vi "Main.vi"() -> ()   [LabVIEW 2013]
doc: "This template is for the Queued Message Handler design pattern.\n\nThe Event Handling Loop generates messages based on user interface actions.\n\nThe Message Handling Loop processes messages generated by the Event Handling Loop, or by other messages. The messages are string values, so new messages can be added easily to the Message Cases case structure in the Message Handling Loop. Each message cluster can also provide an optional value for Message Data, which is a variant that can be converted to whatever message-specific data is required."
uses:
  controls/UI Data.ctl
  <vilib>/vision/Image Controls.llb/IMAQ Image.ctl
  support/Message Queue/Message Queue.lvlib
  support/User Event - Stop/User Event - Stop.lvlib
  support/FPGA/FPGA Frame Grabbing.lvlib
  <vilib>/vision/NI_Vision_Development_Module.lvlib
  support/Image Processing/Image Processing.lvlib
panel:
  out "Wingbeat Amplitude Graph":dynamicdata(graph)
  in  "Stop Charts":bool
  in  "NumWingSectors":u8=12
  in  "Wing ROIs":T1
  out "combo mask":T2(plugin-control)
  out "right \nannulus":T3={"Center X"=1090, "Center Y"=659, "Inner Radius"=200, "Outer Radius"=405, "Start Angle"=0.0, "End Angle"=90.0} {"End Angle" format="%.2f"; "Start Angle" format="%.2f"; "Center X" scale=0.0..1024.0}
  out "right masked image":T2(plugin-control)
  out "right mask":T2(plugin-control)
  out "left annulus":T3={"Center X"=929, "Center Y"=663, "Inner Radius"=200, "Outer Radius"=405, "Start Angle"=90.0, "End Angle"=180.0} {"End Angle" format="%.2f"; "Start Angle" format="%.2f"; "Center X" scale=0.0..1024.0}
  out "left masked image":T2(plugin-control)
  out "left mask":T2(plugin-control)
  in  "Accept Threshold":bool
  in  "Threshold Range":cluster{"Lower value":dbl, "Upper value":dbl}={"Lower value"=106.82432432432432, "Upper value"=255.0} {"Upper value" min=0.0 max=255.0 scale=0.0..255.0; "Lower value" min=0.0 max=255.0 scale=0.0..255.0}
  out "FPGA image info":T6={"Image Type"=0, "Unit"=enum."Undefined", "X Resolution"=2040, "Y Resolution"=1088, "X Step"=1.0, "Y Step"=1.0, "Image Name"="Image"} {"Image Type" items=["Grayscale (U8)", "Grayscale (I16)", "Grayscale (SGL)", "Complex (CSG)", "RGB (U32)", "HSL (U32)", "RGB (U64)", "Grayscale (U16)"]}
  out "Processed Image":T2(plugin-control)
  in  "Stream?":bool
  out "FPGA Image":T2(plugin-control)
  in  "Save Mask Coordinates":bool
  in  "Test Visual Response":bool
  in  "Test FPGA":bool
  out "Status Update":string="VI Stopped"
  in  "Define Mask":bool
  in  "Acquire Image":bool
  in  "Stop":bool
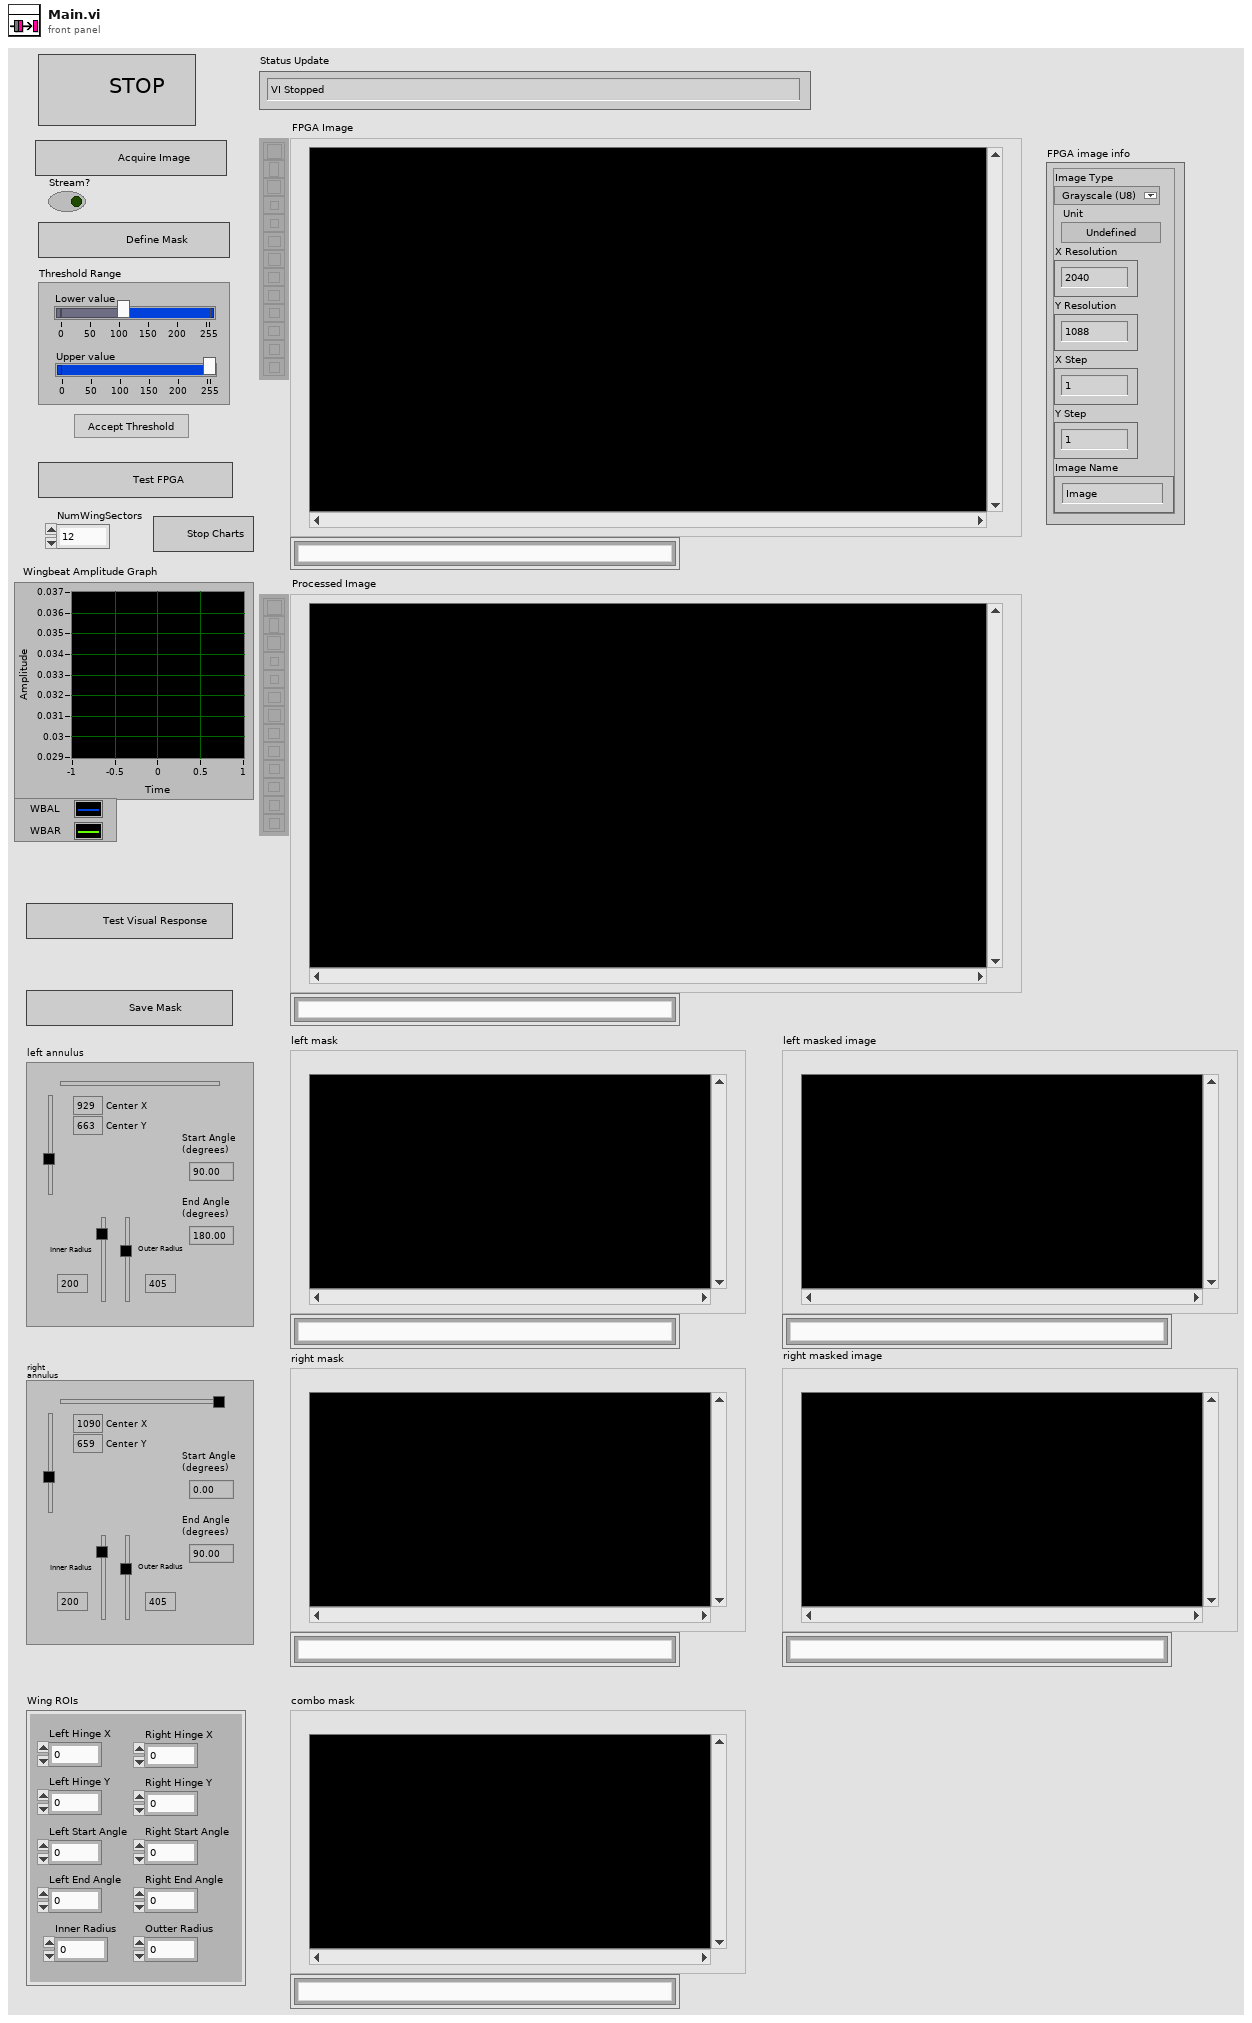
[diagram p1: front panel]
types:
  T1 = cluster{"Left Hinge X":u16, "Left Hinge Y":u16, "Inner Radius":u16, "Outter Radius":u16, "Right Hinge X":u16, "Right Hinge Y":u16, "Right Start Angle":i16, "Right End Angle":i16, "Left Start Angle":i16, "Left End Angle":i16}
  T2 = typedef "IMAQ Image.ctl" = refnum<image>
  T3 = typedef "IMAQ Circle" = cluster{"Center X":i32, "Center Y":i32, "Inner Radius":i32, "Outer Radius":i32, "Start Angle":dbl, "End Angle":dbl}
  T4 = typedef "Image Type" = u32
  T5 = typedef "Image Unit" = enum32{"Undefined", "Angström", "Micrometer", "Millimeter", "Centimeter", "Meter", "Kilometer", "Microinch", "Inch", "Feet", "Nautical miles", "Standard miles", "Steps"}
  T6 = cluster{"Image Type":T4, "Unit":T5, "X Resolution":i32, "Y Resolution":i32, "X Step":sgl, "Y Step":sgl, "Image Name":string}
  T7 = typedef "UI Data.ctl" = cluster{"Boolean <Replace Me>":bool, "Initial Message":string, "Numeric <Replace Me>":dbl, "Acquire Image Ref":refnum<vi>, "Define Mask Ref":refnum<vi>, "Status Update Ref":refnum<vi>, "Stop Button Ref":refnum<vi>, "FPGA Image":T2, "Processed Image":T2, "Left Annulus":cluster{"Center X":i32, "Center Y":i32, "Inner Radius":i32, "Outer Radius":i32, "Start Angle":dbl, "End Angle":dbl}, "Right Annulus":cluster{"Center X":i32, "Center Y":i32, "Inner Radius":i32, "Outer Radius":i32, "Start Angle":dbl, "End Angle":dbl}}
  T8 = typedef "Message Queue.lvlib/All Message Queues.ctl" = cluster{"UI":refnum<queue>}
  T9 = cluster{"Center X":i32, "Center Y":i32, "Inner Radius":i32, "Outer Radius":i32, "Start Angle":dbl, "End Angle":dbl}
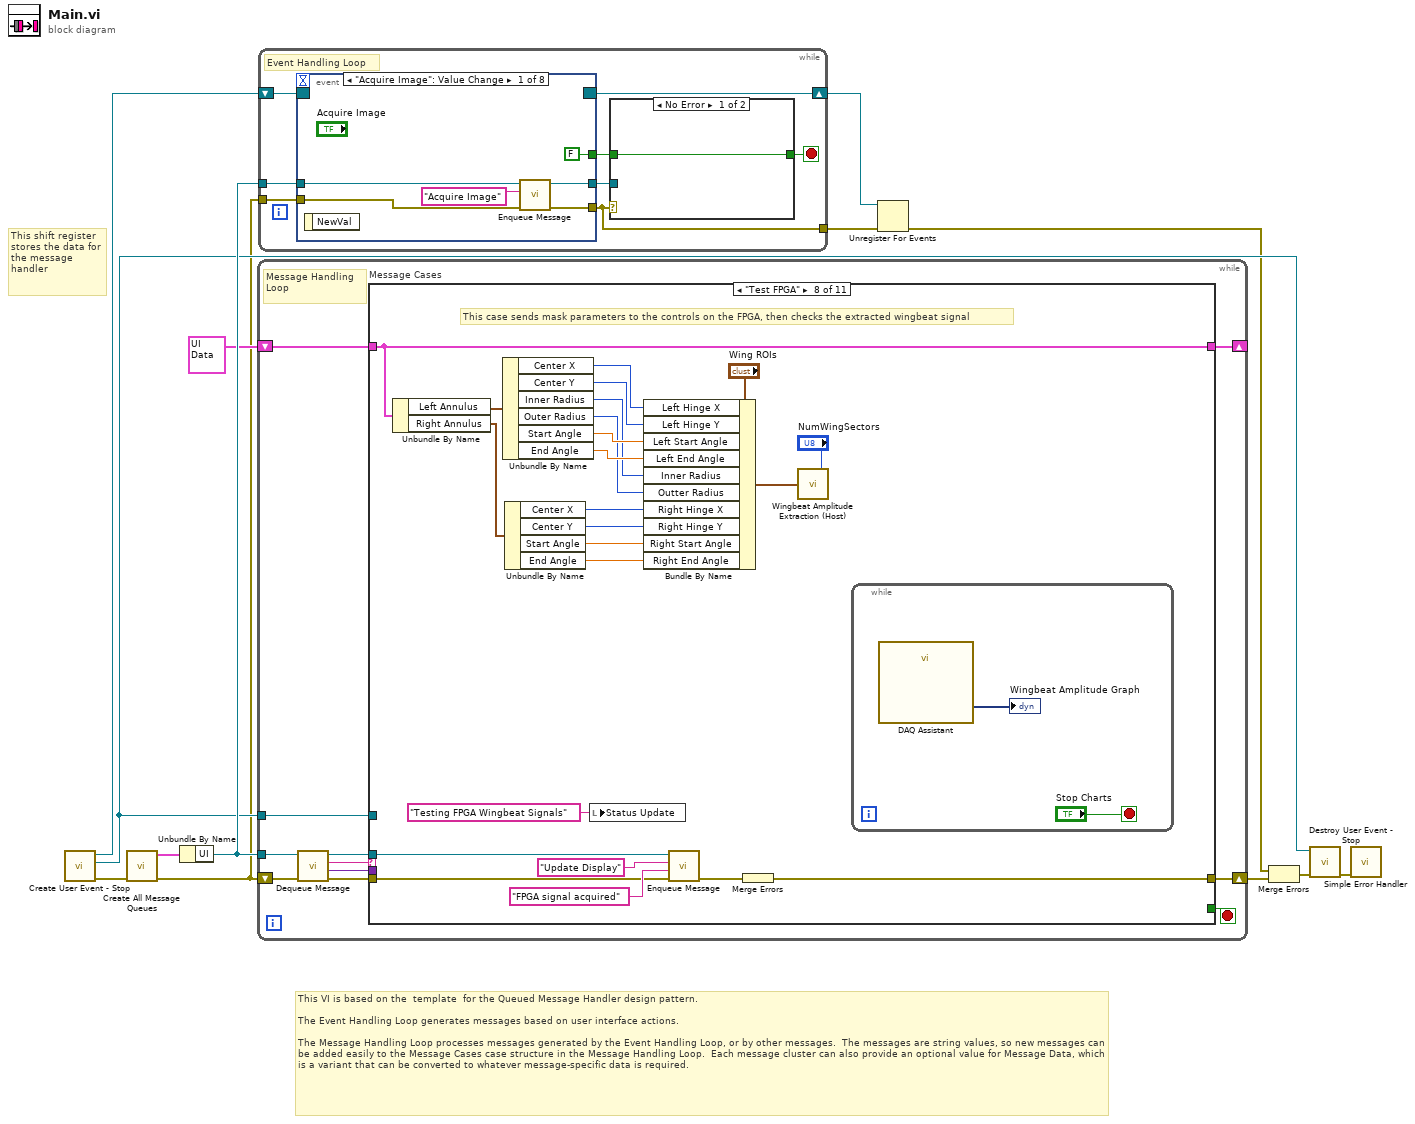
[diagram p0: block diagram]
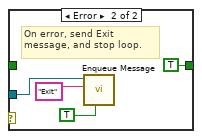
[diagram p2: hidden frame]
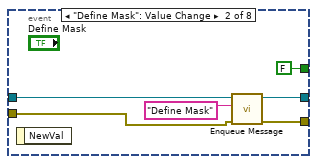
[diagram p3: hidden frame]
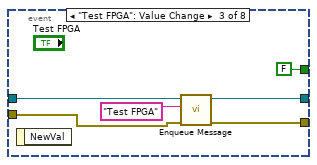
[diagram p4: hidden frame]
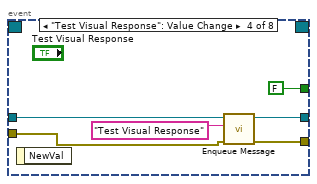
[diagram p5: hidden frame]
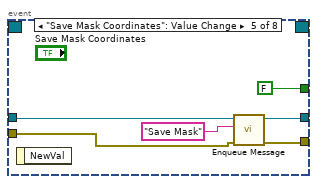
[diagram p6: hidden frame]
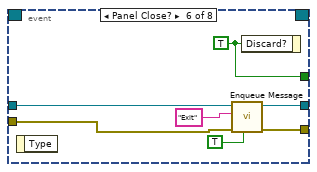
[diagram p7: hidden frame]
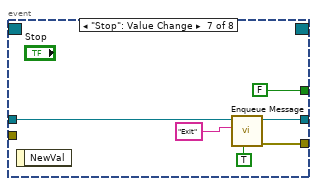
[diagram p8: hidden frame]
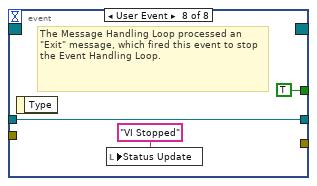
[diagram p9: hidden frame]
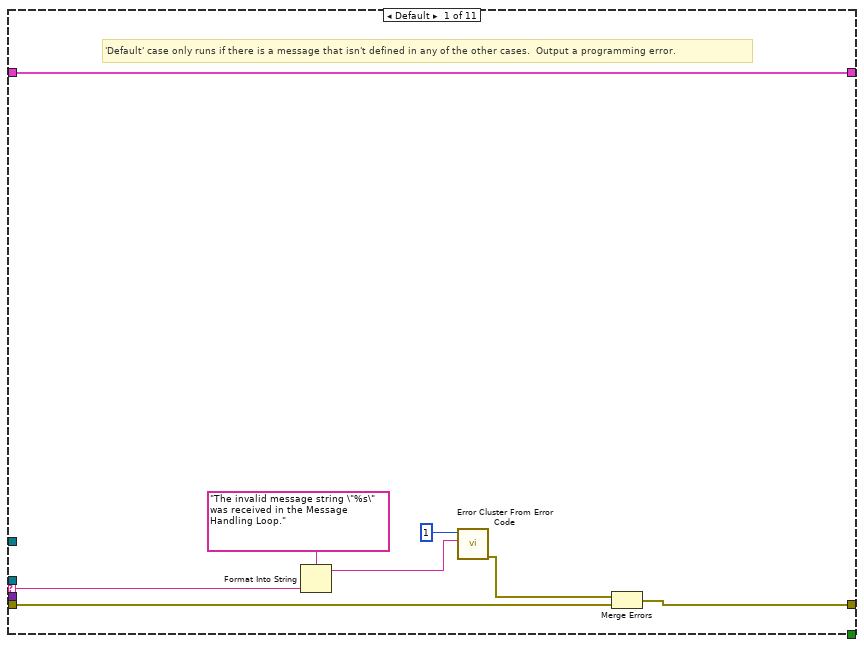
[diagram p10: hidden frame]
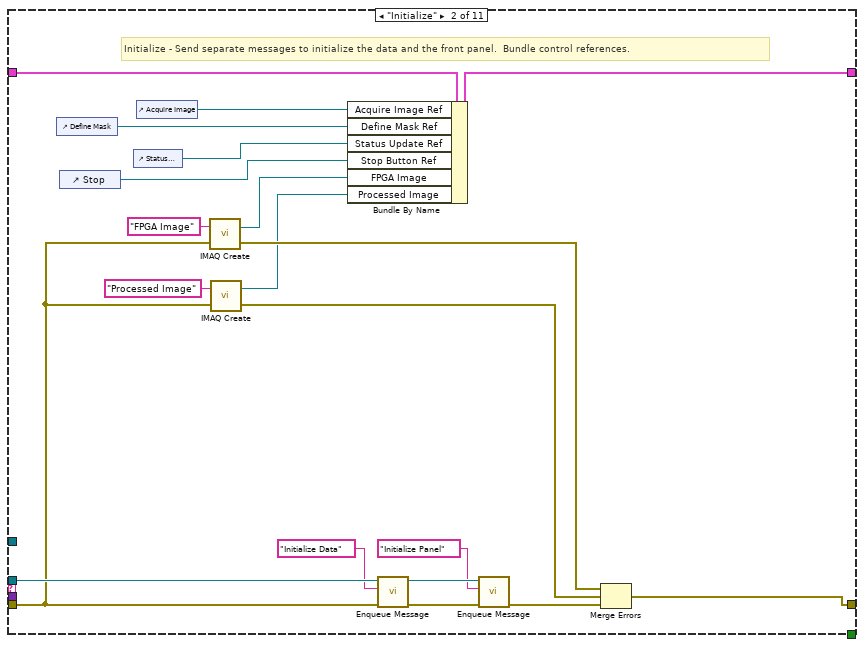
[diagram p11: hidden frame]
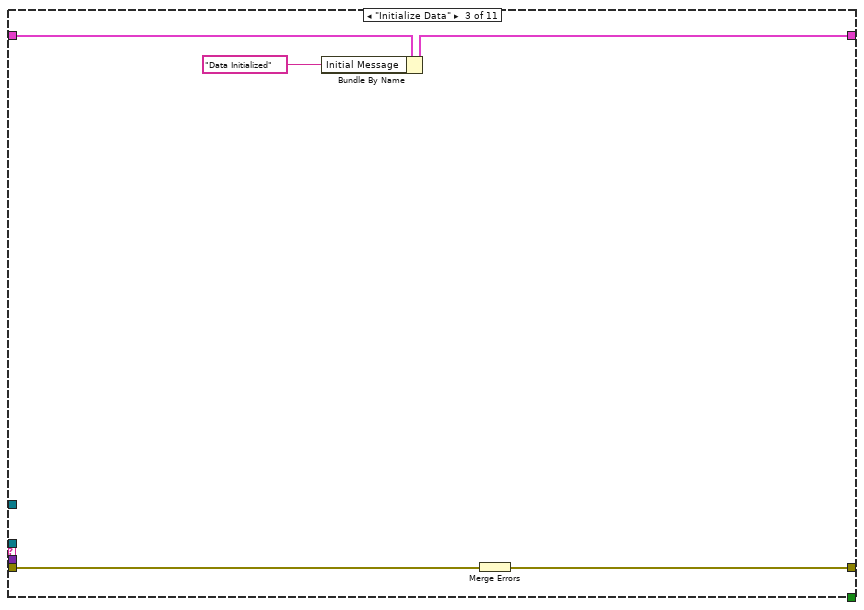
[diagram p12: hidden frame]
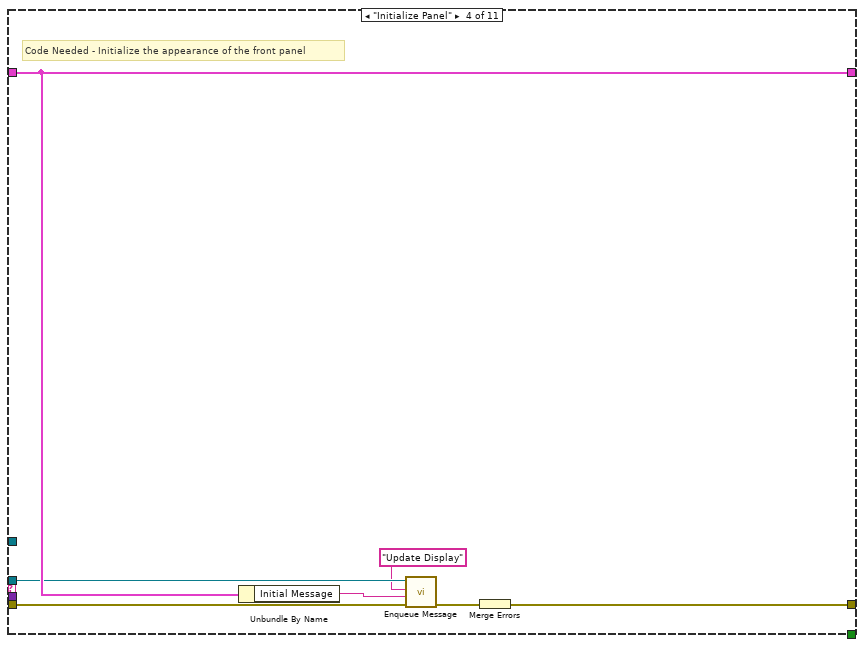
[diagram p13: hidden frame]
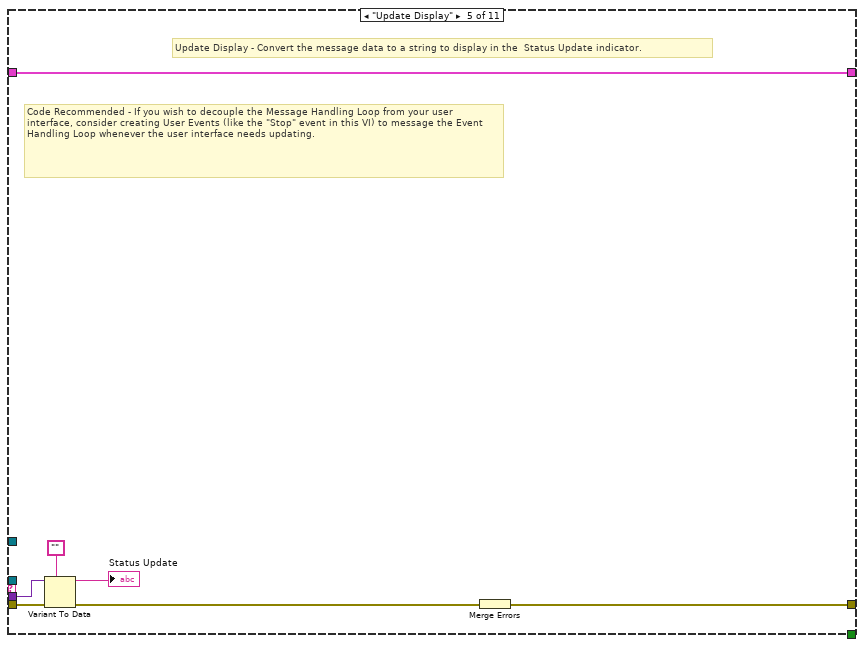
[diagram p14: hidden frame]
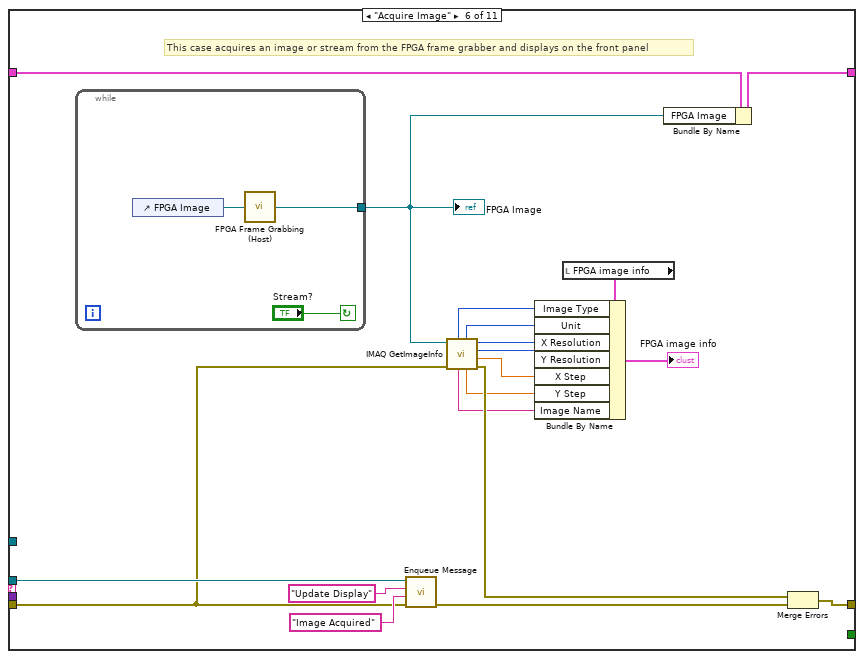
[diagram p15: hidden frame]
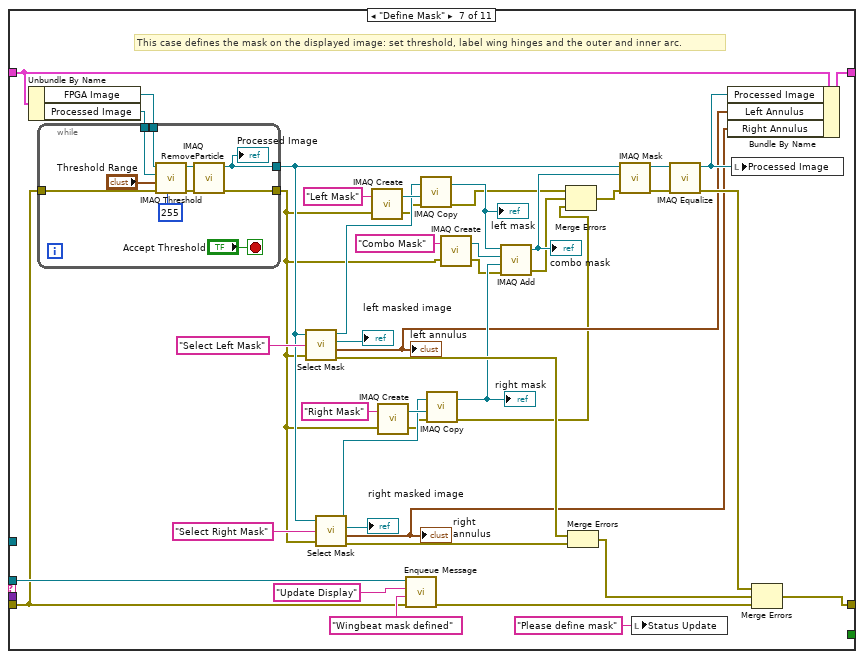
[diagram p16: hidden frame]
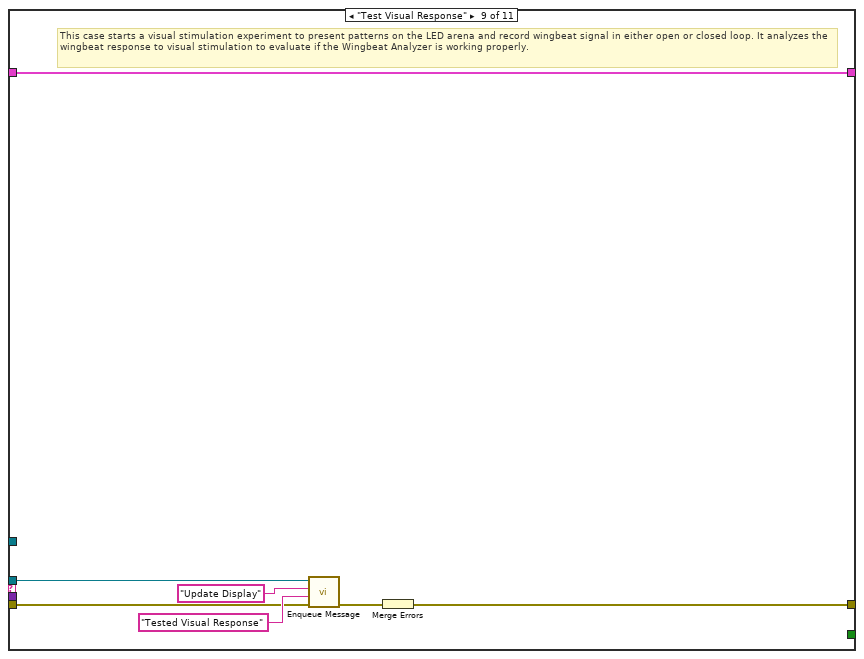
[diagram p17: hidden frame]
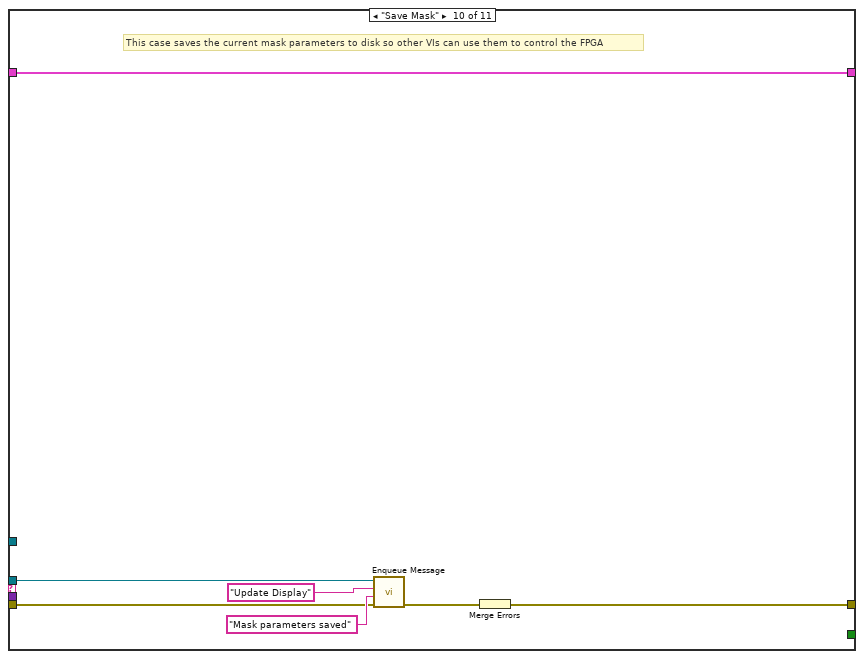
[diagram p18: hidden frame]
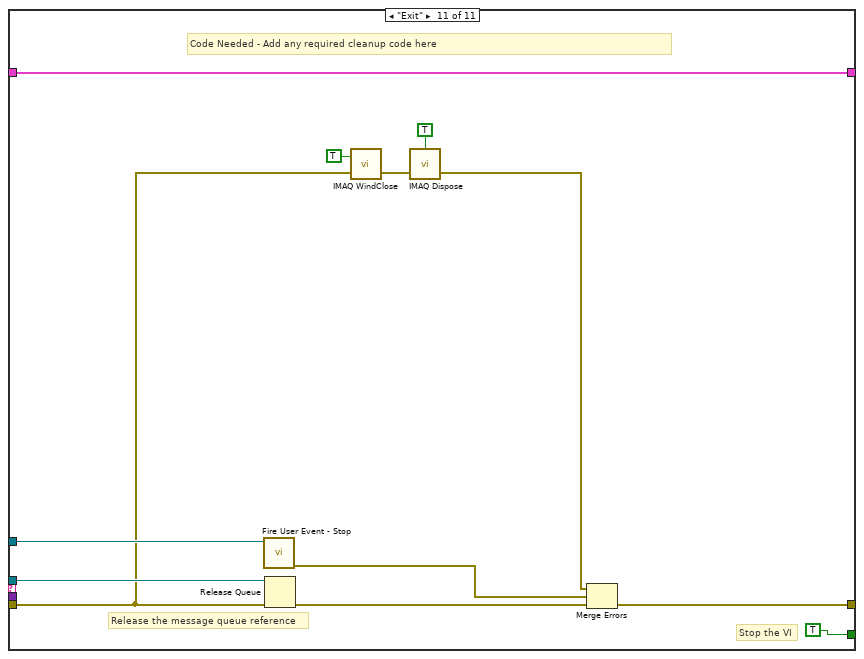
[diagram p19: hidden frame]
diagram:
  # "This VI is based on the  template  for the Queued Message Handler design pattern.\n\nThe Event Handling Loop generates messages based on user interface actions.\n\nThe Message Handling Loop processes messages generated by the Event Handling Loop, or by other messages.  The messages are string values, so new messages can be added easily to the Message Cases case structure in the Message Handling Loop.  Each message cluster can also provide an optional value for Message Data, which is a variant that can be converted to whatever message-specific data is required."
  # "This shift register\nstores the data for the message handler"
  n1 = call "Create User Event - Stop.vi"() -> ("error out"=w9:errorcluster, "User Event - Stop"=w6:refnum<user-event>, "Stop Event Registration Refnum"=w10:refnum<event-registration>)  [unwired: 9 in]
  n2 = call "Create All Message Queues.vi"("error in (no error)"=w9) -> ("error out"=w1:errorcluster, "Message Queues out"=w13:T8)  [unwired: 9 in]
  n3 = Unbundle By Name(w13) -> ("UI"=w11:refnum<queue>)
  n4 = while {
    tunnel: w11 -> [w14]
    shift-right: [w23] -> _
    shift-left: T7 {"Boolean <Replace Me>"=TRUE, "Initial Message"="", "Numeric <Replace Me>"=0.0, "Acquire Image Ref"=refnum, "Define Mask Ref"=refnum, "Status Update Ref"=refnum, "Stop Button Ref"=refnum, "FPGA Image"=refnum, "Processed Image"=refnum, "Left Annulus"={"Center X"=0, "Center Y"=0, "Inner Radius"=0, "Outer Radius"=0, "Start Angle"=0.0, "End Angle"=0.0}, "Right Annulus"={"Center X"=0, "Center Y"=0, "Inner Radius"=0, "Outer Radius"=0, "Start Angle"=0.0, "End Angle"=0.0}} ("Data Cluster") -> [w24]
    tunnel: w6 -> [w20]
    shift-right: [w21] -> w12
    shift-left: w1 -> [w19]
    stop <- w22 stop-if-true
    # "Message Handling Loop"
    n5 = call "Dequeue Message.vi"("error in (no error)"=w19, "Message Queue"=w14) -> ("error out"=w18:errorcluster, "Message Data"=w16:variant, "Message"=w17:string, "dup Message Queue"=w15:refnum<queue>)  [unwired: 6 in]
    n6 = case "Message Cases" shown="\"Test FPGA\"" w17 {
      selector: w17 -> [w30 _ _ _ _ _ _ _ _ _ _]
      tunnel: w15 -> [_ w50 _ w61 _ w88 w137 w166 w174 w182 w198]
      tunnel: w18 -> [w27 w35 w57 w62 w69 w83 w134 w167 w175 w180 w187]
      tunnel: [w25 w37 w53 w63 w70 w90 w94 w165 w173 w185 w194] -> w21
      tunnel: w24 -> [w32 w47 w56 w64 w71 w85 w133 w164 w179 w186 w197]
      tunnel: [w32 w46 w55 w64 w71 w84 w132 w164 w179 w186 w197] -> w23
      tunnel: [_ _ _ _ _ _ _ _ _ _ TRUE] -> w22
      tunnel: w16 -> [_ _ _ _ w68 _ _ _ _ _ _]
      tunnel: w20 -> [_ _ _ _ _ _ _ _ _ _ w193]
      frame Default {
        # "'Default' case only runs if there is a message that isn't defined in any of the other cases.  Output a programming error."
        n7 = Format Into String(format string="The invalid message string \"%s\" was received in the Message Handling Loop." ("Unknown Message Error Text"), w30) -> (resulting string=w28:string)  [unwired: 2 in, 1 out]
        n8 = call <vilib>:"Error Cluster From Error Code.vi"("error message (\"\")"=w28, "error code (0)"=1) -> ("error out"=w26:errorcluster)  [unwired: 7 in]
        n9 = Merge Errors(w26, w27) -> (w25:errorcluster)
      }
      frame "Initialize" {
        # "Initialize - Send separate messages to initialize the data and the front panel.  Bundle control references."
        n10 = control-ref of="Define Mask"() -> (w44:refnum<vi>)
        n11 = control-ref of="Stop"() -> (w42:refnum<vi>)
        n12 = control-ref of="Status Update"() -> (w43:refnum<vi>)
        n13 = control-ref of="Acquire Image"() -> (w45:refnum<vi>)
        n14 = call "IMAQ Create"("Image Name"="FPGA Image", "error in (no error)"=w35) -> ("New Image"=w40:T2, "error out"=w36:errorcluster)  [unwired: 3 in]
        n15 = call "IMAQ Create"("Image Name"="Processed Image", "error in (no error)"=w35) -> ("New Image"=w33:T2, "error out"=w34:errorcluster)  [unwired: 3 in]
        n16 = Bundle By Name(cluster=w47, "Acquire Image Ref"=w45, "Define Mask Ref"=w44, "Status Update Ref"=w43, "Stop Button Ref"=w42, "FPGA Image"=w40, "Processed Image"=w33) -> (w46:T7)
        n17 = call "Enqueue Message.vi"("error in (no error)"=w35, "Message"="Initialize Data", "Message Queue"=w50) -> ("error out"=w52:errorcluster, "dup Message Queue"=w51:refnum<queue>)  [unwired: 7 in]
        n18 = call "Enqueue Message.vi"("error in (no error)"=w52, "Message"="Initialize Panel", "Message Queue"=w51) -> ("error out"=w38:errorcluster)  [unwired: 7 in, 1 out]
        n19 = Merge Errors(w36, w34, w38) -> (w37:errorcluster)
      }
      frame "Initialize Data" {
        n20 = Bundle By Name(cluster=w56, "Initial Message"="Data Initialized") -> (w55:T7)
        n21 = Merge Errors(w57) -> (w53:errorcluster)
      }
      frame "Initialize Panel" {
        # "Code Needed - Initialize the appearance of the front panel"
        n22 = Unbundle By Name(w64) -> ("Initial Message"=w58:string)
        n23 = call "Enqueue Message.vi"("error in (no error)"=w62, "Message Data"=w58, "Message"="Update Display", "Message Queue"=w61) -> ("error out"=w60:errorcluster)  [unwired: 6 in, 1 out]
        n24 = Merge Errors(w60) -> (w63:errorcluster)
      }
      frame "Update Display" {
        # "Code Recommended - If you wish to decouple the Message Handling Loop from your user interface, consider creating User Events (like the \"Stop\" event in this VI) to message the Event Handling Loop whenever the user interface needs updating."
        # "Update Display - Convert the message data to a string to display in the  Status Update indicator."
        n25 = Variant To Data(error in=w69, type="", Variant=w68) -> (data=→"Status Update":string, error out=w66:errorcluster)
        n26 = Merge Errors(w66) -> (w70:errorcluster)
      }
      frame "Acquire Image" {
        # "This case acquires an image or stream from the FPGA frame grabber and displays on the front panel"
        n27 = while {
          tunnel: [w92] -> w72
          stop <- "Stream?" continue-if-true
          n28 = control-ref of="FPGA Image"() -> (w91:refnum<vi>)
          n29 = call "FPGA Frame Grabbing (Host).vi"("Ctl Refnum"=w91) -> ("Image"=w92:T2)
        }
        "FPGA Image" <- w72
        n30 = call "Enqueue Message.vi"("error in (no error)"=w83, "Message Data"="Image Acquired" ("\"Do Something\" button pressed"), "Message"="Update Display", "Message Queue"=w88) -> ("error out"=w89:errorcluster)  [unwired: 6 in, 1 out]
        n31 = call "IMAQ GetImageInfo"("error in (no error)"=w83, "Image"=w72) -> ("error out"=w82:errorcluster, "X Step"=w77:sgl, "Y Resolution"=w78:i32, "X Resolution"=w79:i32, "Y Step"=w76:sgl, "Unit"=w80:T5, "Image Name"=w75:string, "Image Type"=w81:T4)  [unwired: 2 in]
        n32 = local read "FPGA image info"() -> (w73:T6)
        n33 = Bundle By Name(cluster=w73, "Image Type"=w81, "Unit"=w80, "X Resolution"=w79, "Y Resolution"=w78, "X Step"=w77, "Y Step"=w76, "Image Name"=w75) -> (→"FPGA image info":T6)
        n34 = Bundle By Name(cluster=w85, "FPGA Image"=w72) -> (w84:T7)
        n35 = Merge Errors(w82, w89) -> (w90:errorcluster)
      }
      frame "Define Mask" {
        # "This case defines the mask on the displayed image: set threshold, label wing hinges and the outer and inner arc."
        n36 = Unbundle By Name(w133) -> ("FPGA Image"=w131:T2, "Processed Image"=w130:T2)
        n37 = while {
          tunnel: w134 -> [w147]
          tunnel: w131 -> [w146]
          tunnel: w130 -> [w145]
          tunnel: [w138] -> w116
          tunnel: [w140] -> w100
          stop <- "Accept Threshold" stop-if-true
          n38 = call "IMAQ Threshold"("Replace Value"=u8 255, "error in (no error)"=w147, "Range"="Threshold Range", "Image Dst"=w145, "Image Src"=w146) -> ("error out"=w143:errorcluster, "Image Dst Out"=w142:T2)  [unwired: 1 in, 4 out]
          n39 = call "IMAQ RemoveParticle"("error in (no error)"=w143, "Image Src"=w142) -> ("error out"=w140:errorcluster, "Image Dst Out"=w138:T2)  [unwired: 5 in, 3 out]
          "Processed Image" <- w138
        }
        n40 = call "Select Mask.vi"("Read \nImage"=w116, "Prompt"="Select Left Mask", "error in"=w100) -> ("mask"=w109:T2, "Masked \nImage"=→"left masked image":T2, "Annulus"=w105:T3, "error out"=w120:errorcluster)  [unwired: 1 out]
        "left annulus" <- w105
        n41 = call "Select Mask.vi"("Read \nImage"=w116, "Prompt"="Select Right Mask", "error in"=w100) -> ("mask"=w107:T2, "Masked \nImage"=→"right masked image":T2, "Annulus"=w104:T3, "error out"=w119:errorcluster)  [unwired: 1 out]
        "right \nannulus" <- w104
        n42 = call "IMAQ Create"("Image Name"="Left Mask", "error in (no error)"=w100) -> ("New Image"=w112:T2, "error out"=w103:errorcluster)  [unwired: 3 in]
        n43 = call "IMAQ Create"("Image Name"="Right Mask", "error in (no error)"=w100) -> ("New Image"=w110:T2, "error out"=w102:errorcluster)  [unwired: 3 in]
        n44 = call "Enqueue Message.vi"("error in (no error)"=w134, "Message Data"="Wingbeat mask defined" ("\"Do Something Else\" button pressed"), "Message"="Update Display", "Message Queue"=w137) -> ("error out"=w95:errorcluster)  [unwired: 6 in, 1 out]
        n45 = call "IMAQ Copy"("error in (no error)"=w103, "Image Dst"=w112, "Image Src"=w109) -> ("error out"=w99:errorcluster, "Image Dst Out"=w108:T2)  [unwired: 3 in]
        "left mask" <- w108
        n46 = call "IMAQ Copy"("error in (no error)"=w102, "Image Dst"=w110, "Image Src"=w107) -> ("error out"=w97:errorcluster, "Image Dst Out"=w106:T2)  [unwired: 3 in]
        "right mask" <- w106
        n47 = call "IMAQ Create"("Image Name"="Combo Mask", "error in (no error)"=w100) -> ("New Image"=w117:T2, "error out"=w101:errorcluster)  [unwired: 3 in]
        n48 = call "IMAQ Add"("Image Src A"=w108, "Image Dst"=w117, "Image Src B"=w106, "error in (no error)"=w101) -> ("Image Dst Out"=w114:T2, "error out"=w98:errorcluster)  [unwired: 3 in]
        "combo mask" <- w114
        n49 = Merge Errors(w99, w98, w97) -> (w96:errorcluster)
        n50 = Merge Errors(w120, w119) -> (w115:errorcluster)
        n51 = call "IMAQ Mask"("error in (no error)"=w96, "Image Mask"=w114, "Image Src"=w116) -> ("error out"=w125:errorcluster, "Image Dst Out"=w126:T2)  [unwired: 1 in, 1 out]
        n52 = local write "Status Update"("Please define mask" ("Status Update")) -> ()
        n53 = call "IMAQ Equalize"("error in (no error)"=w125, "Image Src"=w126) -> ("error out"=w128:errorcluster, "Image Dst Out"=w124:T2)  [unwired: 4 in, 4 out]
        n54 = Bundle By Name(cluster=w133, "Processed Image"=w124, "Left Annulus"=w105, "Right Annulus"=w104) -> (w132:T7)
        n55 = local write "Processed Image"(w124) -> ()
        n56 = Merge Errors(w128, w115, w95) -> (w94:errorcluster)
      }
      frame "Test FPGA" {
        # "This case sends mask parameters to the controls on the FPGA, then checks the extracted wingbeat signal"
        n57 = Unbundle By Name(w164) -> ("Left Annulus"=w163:T9, "Right Annulus"=w162:T9)
        n58 = Unbundle By Name(w163) -> ("Center X"=w160:i32, "Center Y"=w159:i32, "Inner Radius"=w156:i32, "Outer Radius"=w155:i32, "Start Angle"=w158:dbl, "End Angle"=w157:dbl)
        n59 = Unbundle By Name(w162) -> ("Center X"=w154:i32, "Center Y"=w153:i32, "Start Angle"=w152:dbl, "End Angle"=w151:dbl)
        n60 = local write "Status Update"("Testing FPGA Wingbeat Signals" ("Status Update")) -> ()
        n61 = Bundle By Name(cluster="Wing ROIs", "Left Hinge X"=w160, "Left Hinge Y"=w159, "Left Start Angle"=w158, "Left End Angle"=w157, "Inner Radius"=w156, "Outter Radius"=w155, "Right Hinge X"=w154, "Right Hinge Y"=w153, "Right Start Angle"=w152, "Right End Angle"=w151) -> (w150:T1)
        n62 = call "Enqueue Message.vi"("error in (no error)"=w167, "Message Data"="FPGA signal acquired" ("\"Do Something\" button pressed"), "Message"="Update Display", "Message Queue"=w166) -> ("error out"=w170:errorcluster)  [unwired: 6 in, 1 out]
        n63 = Merge Errors(w170) -> (w165:errorcluster)
        n64 = call "Wingbeat Amplitude Extraction (Host).vi"("NumWingSectors"="NumWingSectors", "Wing ROIs"=w150) -> ()
        n65 = while {
          stop <- "Stop Charts" stop-if-true
          n66 = call "DAQ Assistant"() -> ("data"=→"Wingbeat Amplitude Graph":dynamicdata)  [unwired: 17 in, 2 out]
        }
      }
      frame "Test Visual Response" {
        # "This case starts a visual stimulation experiment to present patterns on the LED arena and record wingbeat signal in either open or closed loop. It analyzes the wingbeat response to visual stimulation to evaluate if the Wingbeat Analyzer is working properly."
        n67 = call "Enqueue Message.vi"("error in (no error)"=w175, "Message Data"="Tested Visual Response" ("\"Do Something\" button pressed"), "Message"="Update Display", "Message Queue"=w174) -> ("error out"=w178:errorcluster)  [unwired: 6 in, 1 out]
        n68 = Merge Errors(w178) -> (w173:errorcluster)
      }
      frame "Save Mask" {
        # "This case saves the current mask parameters to disk so other VIs can use them to control the FPGA"
        n69 = call "Enqueue Message.vi"("error in (no error)"=w180, "Message Data"="Mask parameters saved" ("\"Do Something Else\" button pressed"), "Message"="Update Display", "Message Queue"=w182) -> ("error out"=w181:errorcluster)  [unwired: 6 in, 1 out]
        n70 = Merge Errors(w181) -> (w185:errorcluster)
      }
      frame "Exit" {
        # "Stop the VI"
        # "Release the message queue reference"
        # "Code Needed - Add any required cleanup code here"
        n71 = call "Fire User Event - Stop.vi"("User Event - Stop"=w193) -> ("error out"=w192:errorcluster)  [unwired: 10 in]
        n72 = Release Queue(queue=w198, error in (no error)=w187) -> (error out=w195:errorcluster)  [unwired: 1 in, 2 out]
        n73 = call "IMAQ WindClose"("Close All Windows (False)"=TRUE, "error in (no error)"=w187) -> ("error out"=w189:errorcluster)  [unwired: 4 in]
        n74 = call "IMAQ Dispose"("All Images? (No)"=TRUE, "error in (no error)"=w189) -> ("error out"=w188:errorcluster)  [unwired: 4 in]
        n75 = Merge Errors(w188, w192, w195) -> (w194:errorcluster)
      }
    }
  }
  n76 = while {
    tunnel: w11 -> [w206]
    tunnel: [w202] -> w4
    shift-right: [w200] -> w3
    shift-left: w10 -> [w201]
    tunnel: w1 -> [w199]
    stop <- w204 stop-if-true
    # "Event Handling Loop"
    n77 = event shown="[0] \"Acquire Image\": Value Change" {
      selector: w201 -> [_ _ _ _ _ _ _ _]
      dyn-events: [_ _ _ _ _ _ _ _] -> w200
      timeout: _ -> [_ _ _ _ _ _ _ _]
      tunnel: [FALSE ("Discard?") FALSE ("Discard?") FALSE ("Discard?") FALSE ("Discard?") FALSE ("Discard?") w248 FALSE ("Discard?") TRUE ("Discard?")] -> w205
      tunnel: w206 -> [w217 w223 w229 w234 w239 w247 w254 w257]
      tunnel: [w216 w221 w226 w231 w236 w246 w253 _] -> w202
      tunnel: [w215 w222 w225 w233 w238 w245 w251 w257] -> w203
      tunnel: w199 -> [w213 w219 w227 w230 w237 w242 _ _]
      event "Acquire Image": Value Change {
        n78 = event-data() -> ()  [unwired: 1 in, 1 out]
        n79 = call "Enqueue Message.vi"("error in (no error)"=w213, "Message"="Acquire Image", "Message Queue"=w217) -> ("error out"=w216:errorcluster, "dup Message Queue"=w215:refnum<queue>)  [unwired: 7 in]
      }
      event "Define Mask": Value Change {
        n80 = event-data() -> ()  [unwired: 1 in, 1 out]
        n81 = call "Enqueue Message.vi"("error in (no error)"=w219, "Message"="Define Mask", "Message Queue"=w223) -> ("error out"=w221:errorcluster, "dup Message Queue"=w222:refnum<queue>)  [unwired: 7 in]
      }
      event "Test FPGA": Value Change {
        n82 = event-data() -> ()  [unwired: 1 in, 1 out]
        n83 = call "Enqueue Message.vi"("error in (no error)"=w227, "Message"="Test FPGA", "Message Queue"=w229) -> ("error out"=w226:errorcluster, "dup Message Queue"=w225:refnum<queue>)  [unwired: 7 in]
      }
      event "Test Visual Response": Value Change {
        n84 = event-data() -> ()  [unwired: 1 in, 1 out]
        n85 = call "Enqueue Message.vi"("error in (no error)"=w230, "Message"="Test Visual Response", "Message Queue"=w234) -> ("error out"=w231:errorcluster, "dup Message Queue"=w233:refnum<queue>)  [unwired: 7 in]
      }
      event "Save Mask Coordinates": Value Change {
        n86 = event-data() -> ()  [unwired: 1 in, 1 out]
        n87 = call "Enqueue Message.vi"("error in (no error)"=w237, "Message"="Save Mask", "Message Queue"=w239) -> ("error out"=w236:errorcluster, "dup Message Queue"=w238:refnum<queue>)  [unwired: 7 in]
      }
      event Panel Close? {
        w248 = TRUE ("Discard?")
        n88 = event-data() -> ()  [unwired: 1 in, 1 out]
        n89 = call "Enqueue Message.vi"("Priority Message? (F)"=TRUE, "error in (no error)"=w242, "Message"="Exit", "Message Queue"=w247) -> ("error out"=w246:errorcluster, "dup Message Queue"=w245:refnum<queue>)  [unwired: 6 in]
        n90 = event-data("Discard?"=w248) -> ()  [unwired: 1 in, 1 out]
      }
      event "Stop": Value Change {
        n91 = event-data() -> ()  [unwired: 1 in, 1 out]
        n92 = call "Enqueue Message.vi"("Priority Message? (F)"=TRUE, "Message"="Exit", "Message Queue"=w254) -> ("error out"=w253:errorcluster, "dup Message Queue"=w251:refnum<queue>)  [unwired: 7 in]
      }
      event User Event {
        # "The Message Handling Loop processed an \"Exit\" message, which fired this event to stop the Event Handling Loop."
        n93 = event-data() -> ()  [unwired: 1 in, 1 out]
        n94 = local write "Status Update"("VI Stopped" ("VI Stopped")) -> ()
      }
    }
    n95 = case shown="No Error" w202 {
      tunnel: [w207 TRUE ("Discard?")] -> w204
      tunnel: w205 -> [w207 _]
      tunnel: w203 -> [_ w210]
      frame No Error {
      }
      frame Error {
        # "On error, send Exit message, and stop loop."
        n96 = call "Enqueue Message.vi"("Priority Message? (F)"=TRUE, "Message"="Exit", "Message Queue"=w210) -> ()  [unwired: 7 in, 2 out]
      }
    }
  }
  n97 = Unregister For Events(event registration refnum=w3, error in=w4) -> (error out=w5:errorcluster)
  n98 = Merge Errors(w5, w12) -> (w7:errorcluster)
  n99 = call "Destroy User Event - Stop.vi"("error in (no error)"=w7, "User Event - Stop"=w6) -> ("error out"=w8:errorcluster)  [unwired: 9 in]
  n100 = call <vilib>:"Simple Error Handler.vi"("error in (no error)"=w8) -> ()  [unwired: 4 in, 5 out]
